vi "Read I64 Direct.vi"(8 "error in (no error)":errorcluster, 11 "CIFTag in":refnum<class "CIF_Iceoryx_Chn_I64.lvclass">) -> (0 "error out":errorcluster, 2 "Data":i64, 3 "CIFTag out":refnum<class "CIF_Iceoryx_Chn_I64.lvclass">)   [LabVIEW 2021, in "CIF_Iceoryx_Chn_I64.lvclass"]
uses:
  CIF_Iceoryx_Chn_I64.lvclass
  D:/dev/Packages/CIF_Channels_Core/src/CIFChannels/CIFChannels.lvclass
  D:/dev/Packages/CIF_Channels_Core/src/Iceorxy_Channels/CIF_Iceoryx_BB/CIF_Iceoryx_BB.lvclass
  CIFChannels/CIFChannels.lvclass/CIFChannels.ctl
  ChannelCommon/typedef/Channel State.ctl
  ChannelCommon/typedef/Direction.ctl
  CIF_Iceoryx_Chn_I64.lvclass/CIF_Iceoryx_Chn_I64.ctl
  CIF_Iceoryx_BB/CIF_Iceoryx_BB.lvclass/CIF_Iceoryx_BB.ctl
  CIFChannels/Accessors/Read Channel State.vi
  CIFChannels/Accessors/Read Direction.vi
  CIFChannels/Accessors/Read Tag Forced.vi
  <vilib>/CIF Foundation/CIF Iceoryx/SubVIs/Get Path.vi
  <vilib>/CIF Foundation/CIF Iceoryx/SubVIs/Convert Error.vi
  <vilib>/CIF Foundation/CIF Iceoryx/Refnum/BB Reader from Refnum.vi
  <vilib>/CIF Foundation/CIF Iceoryx/SubVIs/Convert Error Core.vi
  ChannelCommon/ChannelCommon.lvlib
  ce9ea653-e601-4b72-a689-e71696d71a83.vi
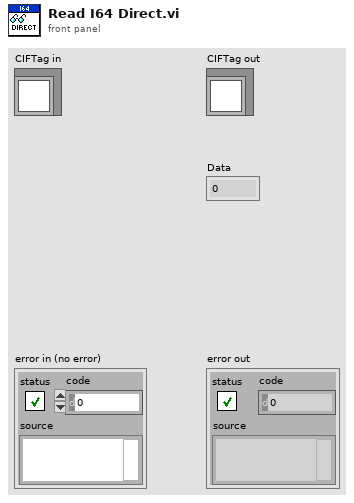
[diagram p1: front panel]
types:
  T1 = typedef "ChannelCommon.lvlib/Channel State.ctl" = enum8{"Creating", "Disconnected", "Connecting", "Connected", "Destroyed"}
  T2 = typedef "ChannelCommon.lvlib/Direction.ctl" = enum8{"Publisher", "Subscriber"}
  T3 = typedef "Iceoryx.lvlib/BB Reader Refnum.ctl" = cluster{"refnum":u64, "BB Reader":enum8{"bb_reader"}}
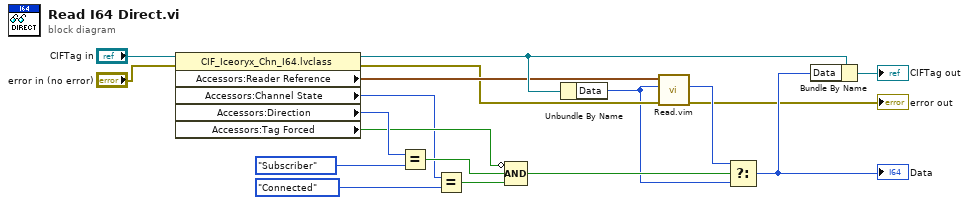
[diagram p0: block diagram]
diagram:
  n1 = property class="CIF_Iceoryx_Chn_I64.lvclass"(reference="CIFTag in", error in="error in (no error)") -> (reference out=w11:refnum<class "CIF_Iceoryx_Chn_I64.lvclass">, error out=w9:errorcluster, "Accessors:Reader Reference"=w10:T3, "Accessors:Channel State"=w12:T1, "Accessors:Direction"=w18:T2, "Accessors:Tag Forced"=w13:bool)
  n2 = Equal?(x=w18, y=Direction."Subscriber") -> (x = y?=w14:bool)
  n3 = Equal?(x=w12, y=Channel_State."Connected") -> (x = y?=w15:bool)
  n4 = Compound Arithmetic op=AND(invert w13, w14, w15) -> (w8:bool)
  n5 = Unbundle By Name(w11) -> ("Data"=w6:i64)
  n6 = call "Read.vim"("error in (no error)"=w9, "Data In"=w6, "Reader Reference"=w10) -> ("error out"=→"error out":errorcluster, "Data Out"=w7:i64)  [unwired: 6 in, 1 out]
  n7 = Select(t=w7, s=w8, f=w6) -> (s? t:f=w3:i64)
  "Data" <- w3
  n8 = Bundle By Name(cluster=w11, "Data"=w3) -> (→"CIFTag out":refnum<class "CIF_Iceoryx_Chn_I64.lvclass">)
